vi "update.properties.vi"(8 "error in (no error)":errorcluster, 10 "properties":map{string, string}(c390), 11 "Run in":refnum<class "Run.lvclass">) -> (0 "error out":errorcluster, 3 "Run out":refnum<class "Run.lvclass">)   [LabVIEW 2020, in "Run.lvclass"]
uses:
  Run.lvclass
  Nominal Client/Nominal Client.lvclass
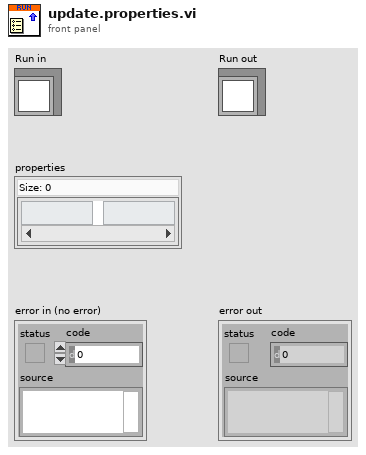
[diagram p1: front panel]
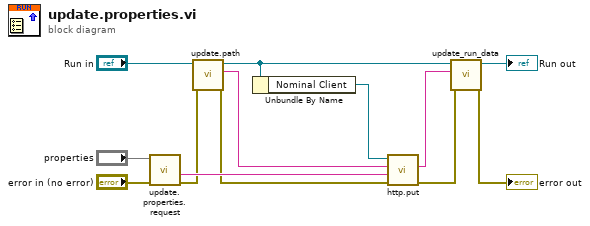
[diagram p0: block diagram]
diagram:
  n1 = call "update.properties.request.vi"("error in"="error in (no error)", "properties"="properties") -> ("error out"=w7:errorcluster, "Request"=w10:string)  [unwired: 8 in]
  n2 = call "update.path.vi"("error in"=w7, "Run"="Run in") -> ("error out"=w6:errorcluster, "path"=w12:string, "Run Out"=w5:refnum<class "Run.lvclass">)  [unwired: 7 in]
  n3 = Unbundle By Name(w5) -> ("Nominal Client"=w11:refnum<class "Nominal Client.lvclass">)
  n4 = call "http.put.vi"("error in"=w6, "Body"=w10, "Path"=w12, "Nominal Client in"=w11) -> ("error out"=w3:errorcluster, "Response"=w4:string)  [unwired: 5 in, 1 out]
  n5 = call "update_run_data.vi"("error in"=w3, "Run JSON"=w4, "Run in"=w5) -> ("error out"=→"error out":errorcluster, "Run out"=→"Run out":refnum<class "Run.lvclass">)  [unwired: 7 in]
